vi "query Swept SA - Trace Values.vi"(8 "error in (no error)":errorcluster, 10 "Trace Index":u32, 11 "Keysight 9020A in":refnum<class "Keysight 9020A.lvclass">) -> (0 "error out":errorcluster, 2 "Trace Values":T1 {"Frequency" format="%#_6p"}, 3 "Keysight 9020A out":refnum<class "Keysight 9020A.lvclass">)   [LabVIEW 2023, in "Spectrum Analyzer.lvlib" / "Keysight 9020A.lvclass"]
uses:
  Keysight 9020A.lvclass
  TYPE DEFINITION/TYPE Trace Value Array.ctl
  Keysight 9020A.lvclass/Keysight 9020A.ctl
  Spectrum Analyzer.lvlib
panel:
  out "size(s)":i32
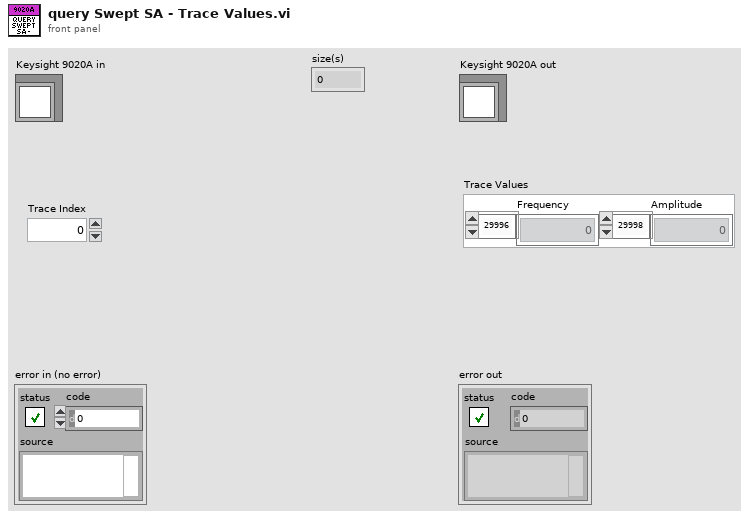
[diagram p1: front panel]
types:
  T1 = typedef "Spectrum Analyzer.lvlib/TYPE Trace Value Array.ctl" = cluster{"Frequency":dbl[], "Amplitude":dbl[]}
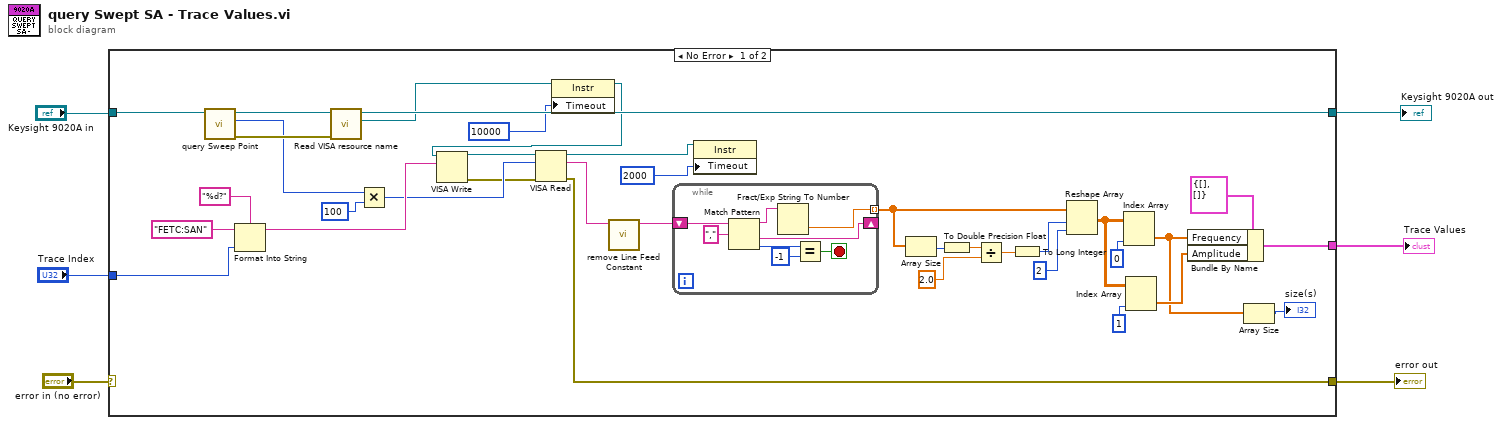
[diagram p0: block diagram]
diagram:
  n1 = case shown="No Error" "error in (no error)" {
    selector: "error in (no error)" -> [_ w51]
    tunnel: "Keysight 9020A in" -> [w25 w52]
    tunnel: [w42 w52] -> w6
    tunnel: [w32 w51] -> w3
    tunnel: "Trace Index" -> [w21 _]
    tunnel: [w26 _] -> w1
    frame No Error {
      n2 = call-dynamic "query Sweep Point.vi"("Keysight 9020A in"=w25) -> ("error out"=w19:errorcluster, "Sweep Point"=w10:u32, "Keysight 9020A out"=w24:refnum<class "Keysight 9020A.lvclass">)  [unwired: 8 in]
      n3 = Format Into String(format string="%d?", initial string="FETC:SAN", w21) -> (resulting string=w20:string)  [unwired: 1 in, 1 out]
      n4 = call "Read VISA resource name.vi"("error in (no error)"=w19, "Keysight 9020A in"=w24) -> ("VISA resource name"=w9:refnum<visa-resource-name>, "Keysight 9020A out"=w42:refnum<class "Keysight 9020A.lvclass">)  [unwired: 7 in, 1 out]
      n5 = Multiply(x=w10, y=u32 100) -> (x*y=w16:u32)
      n6 = property class="Instr"(reference=w9, "Timeout"=u32 10000 ("General Settings:Timeout Value")) -> (reference out=w11:refnum<visa-resource-name>)  [unwired: 1 in, 1 out]
      n7 = VISA Write(VISA resource name=w11, write buffer=w20) -> (VISA resource name out=w17:refnum<visa-resource-name>, error out=w15:errorcluster)  [unwired: 1 in, 1 out]
      n8 = VISA Read(VISA resource name=w17, byte count=w16, error in (no error)=w15) -> (VISA resource name out=w8:refnum<visa-resource-name>, read buffer=w41:string, error out=w32:errorcluster)  [unwired: 1 out]
      n9 = call "remove Line Feed Constant.vi"("Input String"=w41) -> ("Line Feed Removed String"=w33:string)  [unwired: 10 in]
      n10 = while {
        shift-right: [w46] -> _
        shift-left: w33 -> [w50]
        tunnel: [w47] -> w40 mode=indexing
        stop <- w43 stop-if-true
        n11 = Match Pattern(string=w50, regular expression=",") -> (before substring=w48:string, after substring=w46:string, offset past match=w45:i32)  [unwired: 1 in, 1 out]
        n12 = Fract/Exp String To Number(string=w48) -> (number=w47:dbl)  [unwired: 3 in, 1 out]
        n13 = Equal?(x=w45, y=-1) -> (x = y?=w43:bool)
      }
      n14 = property class="Instr"(reference=w8, "Timeout"=u32 2000 ("General Settings:Timeout Value")) -> ()  [unwired: 1 in, 2 out]
      n15 = Array Size(array=w40) -> (size(s)=w39:i32)
      n16 = To Double Precision Float(number=w39) -> (double precision float=w37:dbl)
      n17 = Divide(x=w37, y=2.0) -> (x/y=w36:dbl)
      n18 = To Long Integer(number=w36) -> (32bit integer=w35:i32)
      n19 = Reshape Array(w40, w35, 2 ("dimension size")) -> (w28:dbl[][])
      n20 = Index Array(array=w28, index (col)=0) -> (element=w14:dbl[])  [unwired: 1 in]
      n21 = Index Array(array=w28, index (col)=1) -> (element=w27:dbl[])  [unwired: 1 in]
      n22 = Bundle By Name(cluster=T1 {"Frequency"=[], "Amplitude"=[]} ("Trace Values 2"), "Frequency"=w14, "Amplitude"=w27) -> (w26:T1)
      n23 = Array Size(array=w14) -> (size(s)=→"size(s)":i32)
    }
    frame Error {
    }
  }
  "error out" <- w3
  "Keysight 9020A out" <- w6
  "Trace Values" <- w1
